vi "Assert Not Equal_Variant.vi"(4 "Execution time (s)":dbl=-1.0, 5 "Assert Only? (F)":bool, 6 "error code (1)":i32=1, 7 "Label":string, 8 "error in (no error)":errorcluster, 9 "Register with caller test (F)":bool, 10 "Y":variant, 11 "X":variant) -> (0 "error out":errorcluster)   [LabVIEW 2020, in "Caraya.lvlib" / "Assert.lvclass"]
doc: "THIS METHOD IS DEPRECATED -- Use \"Assert NotEqual Value and Type_Variant.vi\" in the future.\n\nGenerates an error if the input condition is not met.\n\nThis method compares the inputs after being cast to a Variant.\nAsserts TRUE if either type or value of inputs differ.\nAsserts FALSE otherwise.\n\nex 1: Comparing two input integers of equal value and type will assert FALSE.\n\nex 2: Comparing two integer inputs of equal value but of different type representation (U8 and I32) will assert TRUE."
uses:
  Assert.lvclass
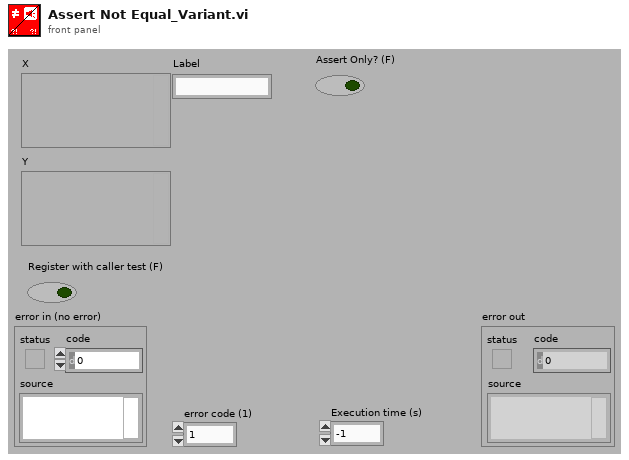
[diagram p1: front panel]
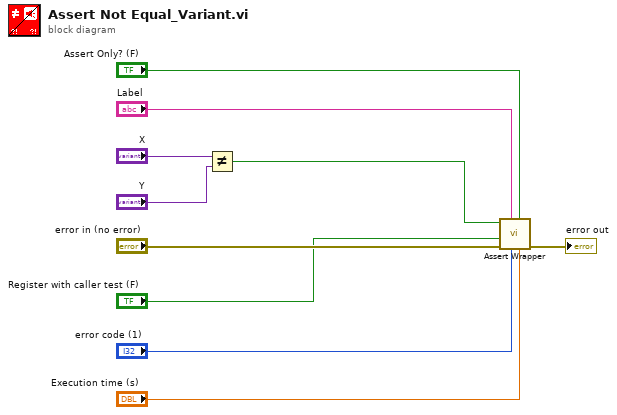
[diagram p0: block diagram]
diagram:
  n1 = Not Equal?(x="X", y="Y") -> (x != y?=w6:bool)
  n2 = call "Assert Wrapper.vi"("Execution time (s)"="Execution time (s)", "Assert Only? (F)"="Assert Only? (F)", "error code (1)"="error code (1)", "Label"="Label", "error in (no error)"="error in (no error)", "Register with caller test (F)"="Register with caller test (F)", "Assert?"=w6) -> ("error out"=→"error out":errorcluster)  [unwired: 1 in, 3 out]
